vi "UI_Draw_Graph.vi"(0 "Picture":picture, 1 "dt":dbl=0.001, 5 "Plot Rect":T2={"left"=96, "top"=648, "right"=1380, "bottom"=896}, 7 "Data":dbl[][](array[numeric]), 9 "Channels":T1(array[cluster]), 11 "error in":errorcluster) -> (4 "New Picture":picture, 15 "error out":errorcluster)   [LabVIEW 2026]
doc: "Channels[i].Graph = True 인 채널만 Plot Rect에 꺾은선 그래프로 그림(Y 자동 스케일, 눈금, 범례, 시간축)."
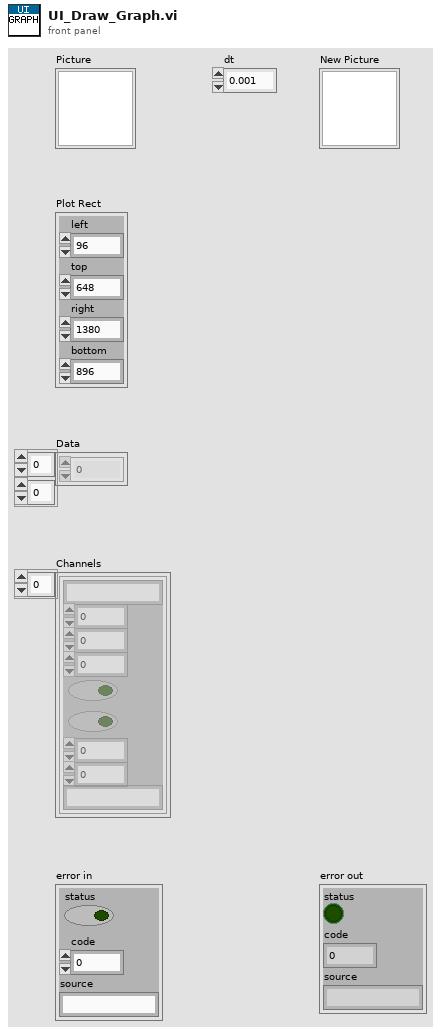
[diagram p1: front panel]
types:
  T1 = cluster{"Name":string, "Value":dbl, "High Limit":dbl, "Low Limit":dbl, "Save":bool, "Graph":bool, "Scale Min":dbl, "Scale Max":dbl, "Unit":string}[]
  T2 = cluster{"left":i16, "top":i16, "right":i16, "bottom":i16}
  T3 = cluster{"Font Name:":string, "Size":i16, "Strikeout?":bool, "Italic?":bool, "Underline?":bool, "Outline?":bool, "Shadow?":bool, "Bold?":bool}
  T4 = enum16{"User-specified Font", "Application Font", "System Font", "Dialog Font"}
  T5 = cluster{"horizontal":enum16{"left", "center", "right"}, "vertical":enum16{"top", "center", "bottom"}}
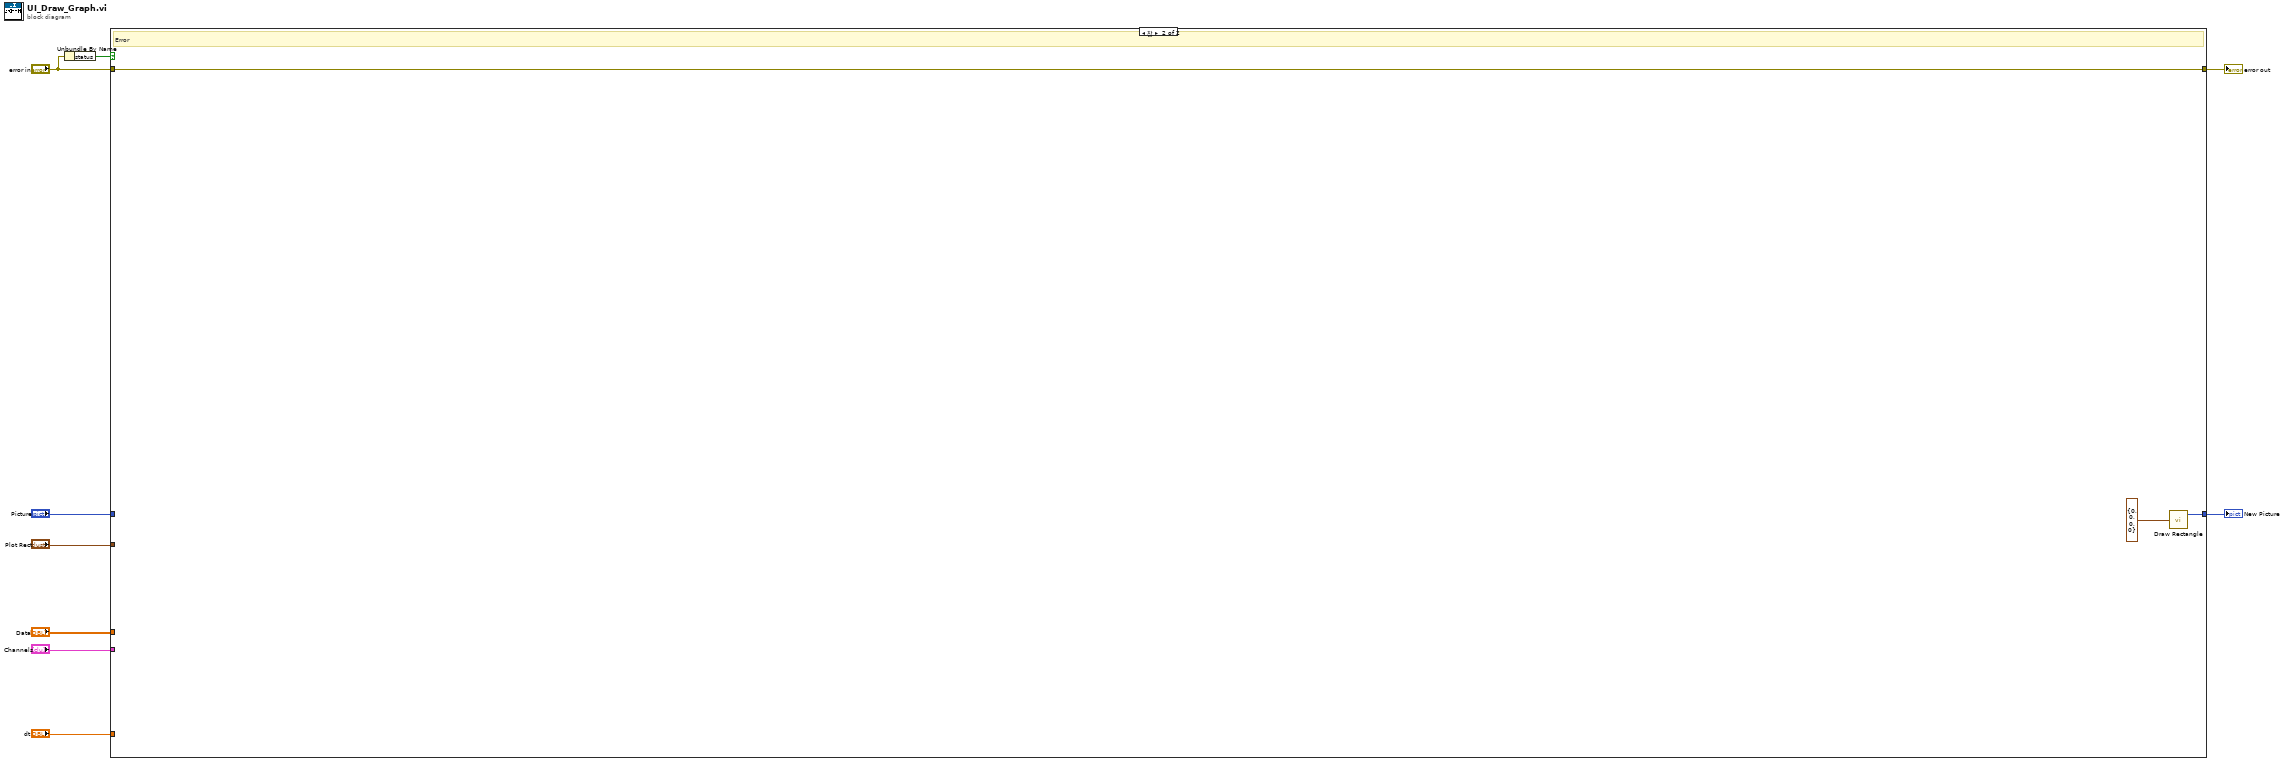
[diagram p0: block diagram]
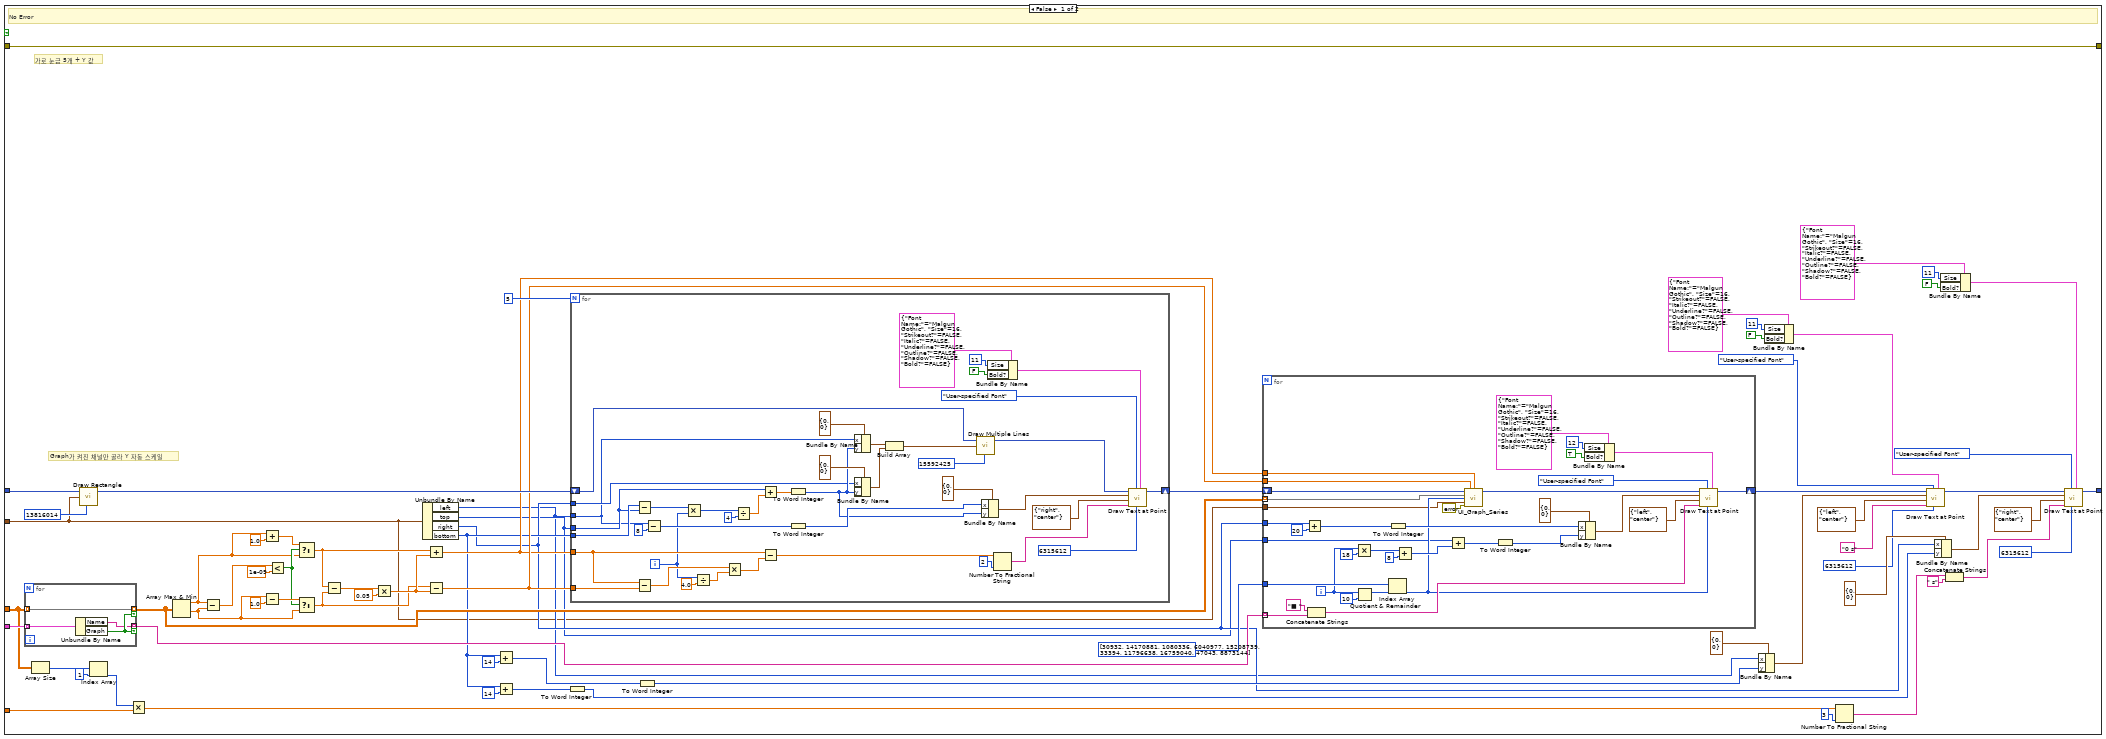
[diagram p2: hidden frame]
diagram:
  n1 = Unbundle By Name("error in") -> ("status"=w7:bool)
  n2 = case shown="참" w7 {
    tunnel: "Picture" -> [w10 _]
    tunnel: "Plot Rect" -> [w11 _]
    tunnel: "Data" -> [w12 _]
    tunnel: "Channels" -> [w13 _]
    tunnel: "dt" -> [w14 _]
    tunnel: "error in" -> [w15 w159]
    tunnel: [w15 w159] -> w9
    tunnel: [w78 w161] -> w8
    frame False {
      # "가로 눈금 5개 + Y 값"
      # "Graph가 켜진 채널만 골라 Y 자동 스케일"
      # "No Error"
      n3 = for {
        tunnel: w12 -> [w155] mode=indexing
        tunnel: w13 -> [w156] mode=indexing
        tunnel: [w155] -> w20 mode=indexing if=w158
        tunnel: [w157] -> w21 mode=indexing if=w158
        n4 = Unbundle By Name(w156) -> ("Name"=w157:string, "Graph"=w158:bool)
      }
      n5 = Array Size(array=w12) -> (size(s)=w44:i32[])
      n6 = call <vilib>:"Draw Rectangle.vi"("picture"=w10, "rect"=w11, "color(black)"=u32 13816014) -> ("new picture"=w39:picture)  [unwired: 6 in]
      n7 = Index Array(array=w44, index=1) -> (element=w46:i32)
      n8 = Multiply(x=w46, y=w14) -> (x*y=w47:dbl)
      n9 = Array Max & Min(array=w20) -> (max value=w22:dbl, min value=w23:dbl)  [unwired: 2 out]
      n10 = Subtract(x=w22, y=w23) -> (x-y=w24:dbl)
      n11 = Add(x=w22, y=1.0) -> (x+y=w28:dbl)
      n12 = Subtract(x=w23, y=1.0) -> (x-y=w31:dbl)
      n13 = Less?(x=w24, y=1e-09) -> (x < y?=w26:bool)
      n14 = Select(t=w28, s=w26, f=w22) -> (s? t:f=w29:dbl)
      n15 = Select(t=w31, s=w26, f=w23) -> (s? t:f=w32:dbl)
      n16 = Subtract(x=w29, y=w32) -> (x-y=w33:dbl)
      n17 = Multiply(x=w33, y=0.05) -> (x*y=w35:dbl)
      n18 = Unbundle By Name(w11) -> ("left"=w16:i16, "top"=w17:i16, "right"=w18:i16, "bottom"=w19:i16)
      n19 = Add(x=w29, y=w35) -> (x+y=w36:dbl)
      n20 = Subtract(x=w32, y=w35) -> (x-y=w37:dbl)
      n21 = Add(x=w19, y=i16 14) -> (x+y=w54:i16)
      n22 = Add(x=w19, y=i16 14) -> (x+y=w67:i16)
      n23 = To Word Integer(number=w67) -> (16bit integer=w68:i16)
      n24 = for {
        N: 5 -> [_]
        tunnel: w16 -> [w115]
        tunnel: w17 -> [w116]
        tunnel: w18 -> [w117]
        tunnel: w19 -> [w118]
        shift-right: [w154] -> w41
        shift-left: w39 -> [w134]
        tunnel: w37 -> [w119]
        tunnel: w36 -> [w120]
        i -> [w114]
        n25 = Subtract(x=w118, y=w116) -> (x-y=w121:i16)
        n26 = Subtract(x=w120, y=w119) -> (x-y=w135:dbl)
        n27 = Subtract(x=w115, y=i16 8) -> (x-y=w143:i16)
        n28 = Multiply(x=w121, y=w114) -> (x*y=w122:i32)
        n29 = Divide(x=w114, y=4.0) -> (x/y=w137:dbl)
        n30 = Multiply(x=w135, y=w137) -> (x*y=w138:dbl)
        n31 = Divide(x=w122, y=4) -> (x/y=w124:dbl)
        n32 = Add(x=w116, y=w124) -> (x+y=w125:dbl)
        n33 = Subtract(x=w120, y=w138) -> (x-y=w139:dbl)
        n34 = To Word Integer(number=w125) -> (16bit integer=w126:i16)
        n35 = To Word Integer(number=w143) -> (16bit integer=w144:i16)
        n36 = Bundle By Name(cluster=cluster{"x":i16, "y":i16} {"x"=0, "y"=0}, "x"=w115, "y"=w126) -> (w128:cluster{"x":i16, "y":i16})
        n37 = Bundle By Name(cluster=cluster{"x":i16, "y":i16} {"x"=0, "y"=0}, "x"=w117, "y"=w126) -> (w130:cluster{"x":i16, "y":i16})
        n38 = Build Array(w128, w130) -> (w131:cluster{"x":i16, "y":i16}[])
        n39 = call <vilib>:"Draw Multiple Lines.vi"("picture"=w134, "line endpoints"=w131, "color(black)"=u32 15592425) -> ("new picture"=w133:picture)  [unwired: 6 in]
        n40 = Bundle By Name(cluster=cluster{"x":i16, "y":i16} {"x"=0, "y"=0}, "x"=w144, "y"=w126) -> (w149:cluster{"x":i16, "y":i16})
        n41 = Bundle By Name(cluster=T3 {"Font Name:"="Malgun Gothic", "Size"=16, "Strikeout?"=FALSE, "Italic?"=FALSE, "Underline?"=FALSE, "Outline?"=FALSE, "Shadow?"=FALSE, "Bold?"=FALSE}, "Size"=i16 11, "Bold?"=FALSE) -> (w153:T3)
        n42 = Number To Fractional String(number=w139, precision (6)=2) -> (F-format string=w141:string)  [unwired: 2 out]
        n43 = call <vilib>:"Draw Text at Point.vi"("[user-specified font]"=w153, "text color(black)"=u32 6315612, "desired font(Application)"=T4."User-specified Font", "text"=w141, "alignment(left, top)"=T5 {"horizontal"=enum."right", "vertical"=enum."center"}, "origin"=w149, "picture"=w133) -> ("new picture"=w154:picture)  [unwired: 3 in, 1 out]
      }
      n44 = To Word Integer(number=w54) -> (16bit integer=w55:i16)
      n45 = for {
        tunnel: u32[] [30932, 14170881, 1080336, 6040977, 15208739, 33394, 11796638, 16759040, 47043, 8873144] ("Palette") -> [w83]
        tunnel: w11 -> [w80]
        tunnel: w18 -> [w84]
        tunnel: w17 -> [w85]
        tunnel: w20 -> [w86] mode=indexing
        shift-right: [w113] -> w43
        shift-left: w41 -> [w93]
        tunnel: w21 -> [w87] mode=indexing
        tunnel: w37 -> [w81]
        tunnel: w36 -> [w82]
        i -> [w79]
        n46 = Add(x=w84, y=i16 20) -> (x+y=w102:i16)
        n47 = Concatenate Strings("■ ", w87) -> (w100:string)
        n48 = Multiply(x=w79, y=18) -> (x*y=w95:i32)
        n49 = Quotient & Remainder(x=w79, y=10) -> (x-y*floor(x/y)=w89:i32)  [unwired: 1 out]
        n50 = Index Array(array=w83, index=w89) -> (element=w90:u32)
        n51 = To Word Integer(number=w102) -> (16bit integer=w103:i16)
        n52 = Add(x=w95, y=8) -> (x+y=w97:i32)
        n53 = Add(x=w85, y=w97) -> (x+y=w98:i32)
        n54 = call "UI_Graph_Series.vi"("Picture"=w93, "Y Min"=w81, "Y Max"=w82, "Samples"=w86, "Color"=w90, "Plot Rect"=w80, "error in"=errorcluster {"status"=FALSE, "code"=0, "source"=""}) -> ("New Picture"=w92:picture)  [unwired: 7 in, 1 out]
        n55 = To Word Integer(number=w98) -> (16bit integer=w104:i16)
        n56 = Bundle By Name(cluster=cluster{"x":i16, "y":i16} {"x"=0, "y"=0}, "x"=w103, "y"=w104) -> (w108:cluster{"x":i16, "y":i16})
        n57 = Bundle By Name(cluster=T3 {"Font Name:"="Malgun Gothic", "Size"=16, "Strikeout?"=FALSE, "Italic?"=FALSE, "Underline?"=FALSE, "Outline?"=FALSE, "Shadow?"=FALSE, "Bold?"=FALSE}, "Size"=i16 12, "Bold?"=TRUE) -> (w112:T3)
        n58 = call <vilib>:"Draw Text at Point.vi"("[user-specified font]"=w112, "text color(black)"=w90, "desired font(Application)"=T4."User-specified Font", "text"=w100, "alignment(left, top)"=T5 {"horizontal"=enum."left", "vertical"=enum."center"}, "origin"=w108, "picture"=w92) -> ("new picture"=w113:picture)  [unwired: 3 in, 1 out]
      }
      n59 = Bundle By Name(cluster=cluster{"x":i16, "y":i16} {"x"=0, "y"=0}, "x"=w16, "y"=w55) -> (w60:cluster{"x":i16, "y":i16})
      n60 = Bundle By Name(cluster=T3 {"Font Name:"="Malgun Gothic", "Size"=16, "Strikeout?"=FALSE, "Italic?"=FALSE, "Underline?"=FALSE, "Outline?"=FALSE, "Shadow?"=FALSE, "Bold?"=FALSE}, "Size"=i16 11, "Bold?"=FALSE) -> (w64:T3)
      n61 = Number To Fractional String(number=w47, precision (6)=3) -> (F-format string=w49:string)  [unwired: 2 out]
      n62 = call <vilib>:"Draw Text at Point.vi"("[user-specified font]"=w64, "text color(black)"=u32 6315612, "desired font(Application)"=T4."User-specified Font", "text"="0 s", "alignment(left, top)"=T5 {"horizontal"=enum."left", "vertical"=enum."center"}, "origin"=w60, "picture"=w43) -> ("new picture"=w65:picture)  [unwired: 3 in, 1 out]
      n63 = Bundle By Name(cluster=cluster{"x":i16, "y":i16} {"x"=0, "y"=0}, "x"=w18, "y"=w68) -> (w73:cluster{"x":i16, "y":i16})
      n64 = Bundle By Name(cluster=T3 {"Font Name:"="Malgun Gothic", "Size"=16, "Strikeout?"=FALSE, "Italic?"=FALSE, "Underline?"=FALSE, "Outline?"=FALSE, "Shadow?"=FALSE, "Bold?"=FALSE}, "Size"=i16 11, "Bold?"=FALSE) -> (w77:T3)
      n65 = Concatenate Strings(w49, " s") -> (w51:string)
      n66 = call <vilib>:"Draw Text at Point.vi"("[user-specified font]"=w77, "text color(black)"=u32 6315612, "desired font(Application)"=T4."User-specified Font", "text"=w51, "alignment(left, top)"=T5 {"horizontal"=enum."right", "vertical"=enum."center"}, "origin"=w73, "picture"=w65) -> ("new picture"=w78:picture)  [unwired: 3 in, 1 out]
    }
    frame True {
      # "Error"
      n67 = call <vilib>:"Draw Rectangle.vi"("rect"=T2 {"left"=0, "top"=0, "right"=0, "bottom"=0}) -> ("new picture"=w161:picture)  [unwired: 8 in]
    }
  }
  "New Picture" <- w8
  "error out" <- w9
